vi "CIF Publish.vi"(6 "CIF Publish Advanced":T2={"Offset"=0, "Length"=-1}, 7 "CIF Channel Header Publisher":T3, 8 "error in (no error)":errorcluster, 9 "Timeout ms":u32, 10 "Data In":u8[](array[numeric]), 11 "Publisher Reference":T4 {"refnum" format="%.0x"}) -> (0 "error out":errorcluster, 1 "Timeout":bool, 2 "Data Out":u8[](array[numeric]), 4 "CIF Publisher Stats":T1)   [LabVIEW 2021, in "Iceoryx.lvlib"]
doc: "Publish to an iceoryx CIF pcap queue. This will write to both publisher queues if created. If there is a backpressure queue with a subscriber attached it can block this VI and it will timeout. On timeout no data will be written to either queue. \n\n<B>CIF Channel Header Publisher:</B> Timestamps for the data in TAI and the clock ID. \n<B>Data In:</B> Flattened PCAP formatted data of the correct Link Type. \n<B>Timeout:</B> Timeout in ms if there is a backpressure queue. \n<B>CIF Publish Advanced:</B> Allows copying a subset of the Data In array. This is useful for variable size payloads where a larger buffer is allocated but only the valid data should be passed."
uses:
  Iceoryx.lvlib
  Refnum/Typedef/CIF Publisher Refnum.ctl
  typedef/CIF Channel Header Publisher.ctl
  typedef/CIF Pcap Publish Advanced.ctl
  typedef/CIF Pcap Publisher Stats.ctl
  typedef/CIF Channel Header.ctl
  SubVIs/Convert Error Core.vi
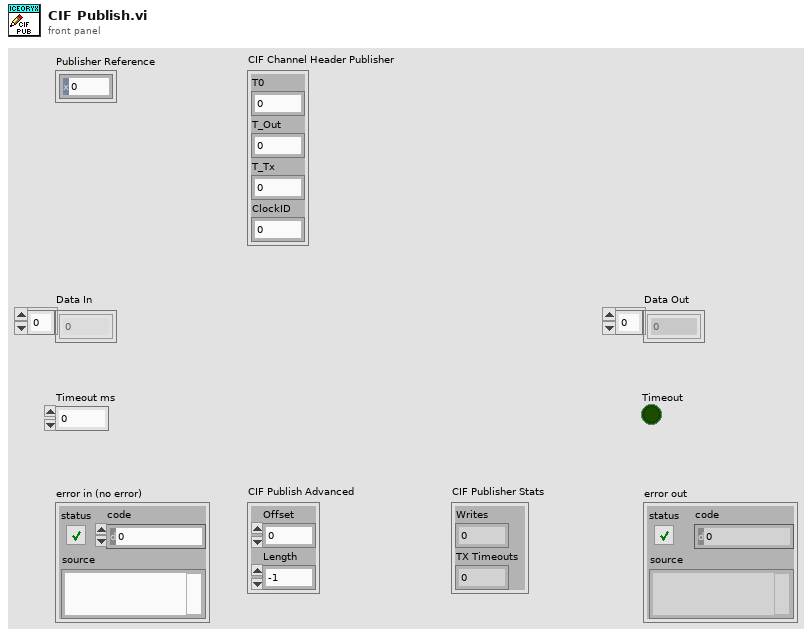
[diagram p1: front panel]
types:
  T1 = typedef "Iceoryx.lvlib/CIF Pcap Publisher Stats.ctl" = cluster{"Writes":u64, "TX Timeouts":u64}
  T2 = typedef "Iceoryx.lvlib/CIF Pcap Publish Advanced.ctl" = cluster{"Offset":u32, "Length":i32}
  T3 = typedef "Iceoryx.lvlib/CIF Channel Header Publisher.ctl" = cluster{"T0":i64, "T_Out":i64, "T_Tx":i64, "ClockID":u8}
  T4 = typedef "Iceoryx.lvlib/CIF Publisher Refnum.ctl" = cluster{"refnum":u64, "CIF Pub":enum8{"cifpub"}}
  T5 = typedef "Iceoryx.lvlib/CIF Channel Header.ctl" = cluster{"Length":u64, "T0":i64, "T_Out":i64, "T_Tx":i64, "Ctr":u64, "ClockID":u8}
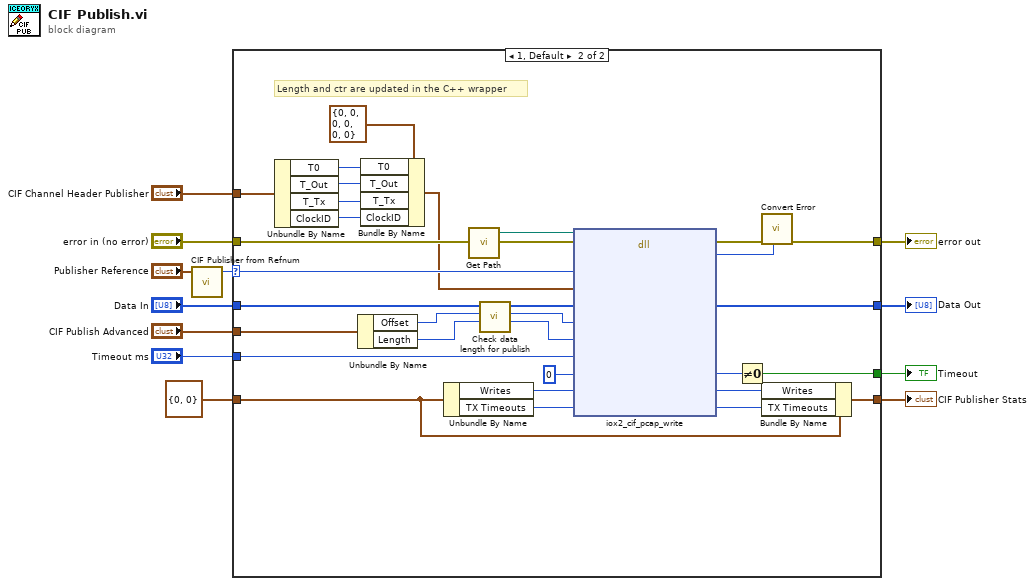
[diagram p0: block diagram]
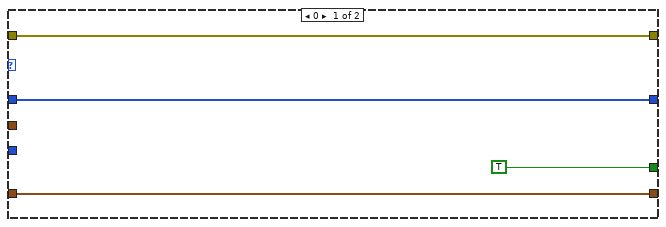
[diagram p2: hidden frame]
diagram:
  n1 = call "CIF Publisher from Refnum.vi"("CIF Publisher Refnum"="Publisher Reference") -> ("CIF Publisher U64"=w1:u64)  [unwired: 4 in]
  n2 = case shown="1, Default" w1 {
    selector: w1 -> [_ w42]
    tunnel: "error in (no error)" -> [w16 w47]
    tunnel: [w16 w43] -> w11
    tunnel: "Timeout ms" -> [_ w41]
    tunnel: [TRUE w39] -> w8
    tunnel: "Data In" -> [w14 w36]
    tunnel: [w14 w37] -> w6
    tunnel: "CIF Channel Header Publisher" -> [_ w31]
    tunnel: "CIF Publish Advanced" -> [_ w28]
    tunnel: [w13 w22] -> w3
    tunnel: T1 {"Writes"=0, "TX Timeouts"=0} ("CIF Publisher Stats") -> [w13 w21]
    frame 0 {
    }
    frame 1, Default {
      # "Length and ctr are updated in the C++ wrapper"
      n3 = Unbundle By Name(w31) -> ("T0"=w32:i64, "T_Out"=w33:i64, "T_Tx"=w34:i64, "ClockID"=w35:u8)
      n4 = Unbundle By Name(w28) -> ("Offset"=w27:u32, "Length"=w26:i32)
      n5 = Bundle By Name(cluster=T5 {"Length"=0, "T0"=0, "T_Out"=0, "T_Tx"=0, "Ctr"=0, "ClockID"=0} ("CIF Channel Header"), "T0"=w32, "T_Out"=w33, "T_Tx"=w34, "ClockID"=w35) -> (w29:T5)
      n6 = Unbundle By Name(w21) -> ("Writes"=w20:u64, "TX Timeouts"=w19:u64)
      n7 = call "Get Path.vi"() -> ("libiox2_cif path"=w46:path)  [unwired: 4 in]
      n8 = call "Check data length for publish.vi"("Length in"=w26, "Offset in"=w27, "Data In"=w36) -> ("Length out"=w18:u32, "Offset out"=w17:u32, "Data out"=w25:u8[])  [unwired: 6 in]
      n9 = dll-call lib="D:/dev/iceoryx2_lvwrapper/dist/iox2_cif.dll" fn="iox2_cif_pcap_write"(path in=w46, error in=w47, "writer"=w42, "header"=w29, "pcap"=w25, "offset"=w17, "length"=w18, "timeout_ms"=w41, "timed_out"=0, "samples"=w20, "timeouts"=w19) -> (error out=w45:errorcluster, "return type"=w44:i32, "pcap"=w37:u8[], "timed_out"=w40:i32, "samples"=w23:u64, "timeouts"=w24:u64)  [unwired: 6 in, 1 out]
      n10 = Not Equal To 0?(x=w40) -> (x != 0?=w39:bool)
      n11 = call "Convert Error.vi"("return type"=w44, "error in (no error)"=w45) -> ("error out"=w43:errorcluster)  [unwired: 9 in]
      n12 = Bundle By Name(cluster=w21, "Writes"=w23, "TX Timeouts"=w24) -> (w22:T1)
    }
  }
  "error out" <- w11
  "Timeout" <- w8
  "Data Out" <- w6
  "CIF Publisher Stats" <- w3
